vi "lab1.vi"() -> ()   [LabVIEW 2025]
panel:
  out "Decoder":bool[][](array[boolean])
  in  "CRC":bool[](array[boolean])
  out "Encoder":bool[][](array[boolean])
  in  "In":bool[](array[boolean])
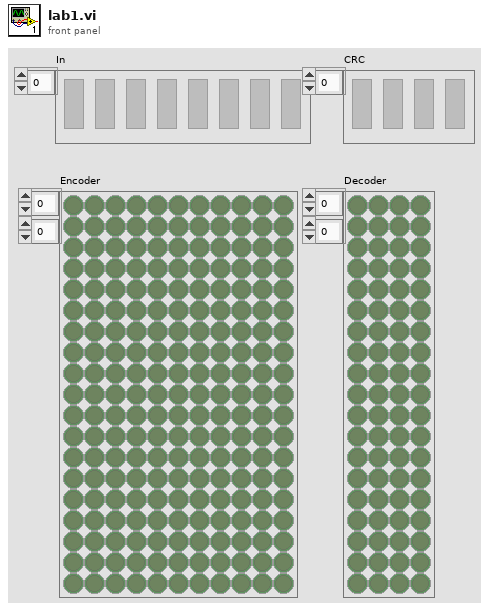
[diagram p1: front panel]
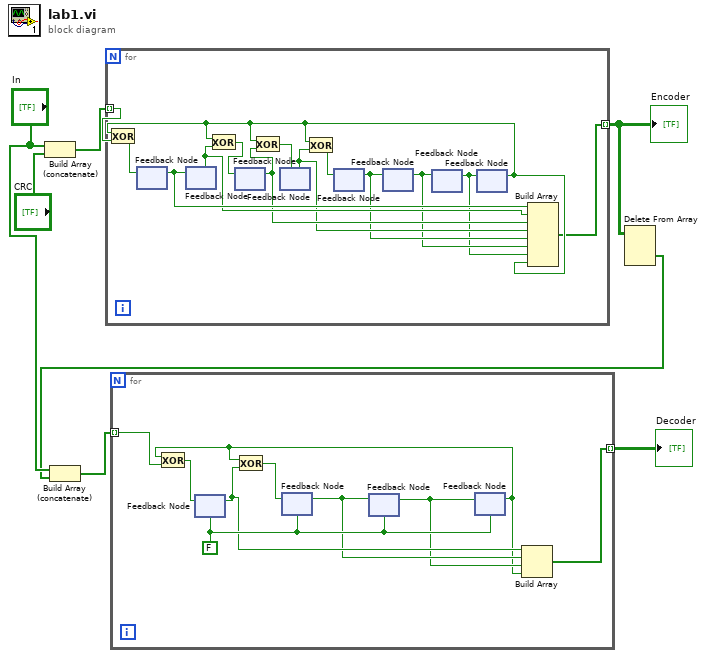
[diagram p0: block diagram]
diagram:
  n1 = Build Array (concatenate)("In", "CRC") -> (w6:bool[])
  n2 = for {
    tunnel: w6 -> [w17] mode=indexing
    tunnel: [w8] -> w2 mode=indexing
    n3 = feedback #1() -> (w16:bool)  [unwired: 1 in]
    n4 = feedback #2() -> (w15:bool)  [unwired: 1 in]
    n5 = feedback-in #2(w16) -> ()
    n6 = feedback #3() -> (w14:bool)  [unwired: 1 in]
    n7 = feedback #4() -> (w13:bool)  [unwired: 1 in]
    n8 = feedback #5() -> (w12:bool)  [unwired: 1 in]
    n9 = feedback #6() -> (w11:bool)  [unwired: 1 in]
    n10 = feedback-in #6(w12) -> ()
    n11 = feedback #7() -> (w10:bool)  [unwired: 1 in]
    n12 = feedback-in #7(w11) -> ()
    n13 = feedback #8() -> (w9:bool)  [unwired: 1 in]
    n14 = Exclusive Or(1:w17, 2:w9) -> (0:w21:bool)
    n15 = feedback-in #1(w21) -> ()
    n16 = Exclusive Or(1:w15, 2:w9) -> (0:w20:bool)
    n17 = feedback-in #3(w20) -> ()
    n18 = Exclusive Or(1:w14, 2:w9) -> (0:w19:bool)
    n19 = feedback-in #4(w19) -> ()
    n20 = Exclusive Or(1:w13, 2:w9) -> (0:w18:bool)
    n21 = feedback-in #5(w18) -> ()
    n22 = feedback-in #8(w10) -> ()
    n23 = Build Array(w16, w15, w14, w13, w12, w11, w10, w9) -> (w8:bool[])
  }
  "Encoder" <- w2
  n24 = Delete From Array(array=w2) -> (deleted portion=w1:bool[])  [unwired: 3 in, 1 out]
  n25 = Build Array (concatenate)("In", w1) -> (w4:bool[])
  n26 = for {
    tunnel: w4 -> [w27] mode=indexing
    tunnel: [w22] -> w5 mode=indexing
    w28 = FALSE
    n27 = feedback #9(w28) -> (w26:bool)
    n28 = feedback #10(w28) -> (w25:bool)
    n29 = feedback #11(w28) -> (w24:bool)
    n30 = feedback-in #11(w25) -> ()
    n31 = feedback #12(w28) -> (w23:bool)
    n32 = Exclusive Or(1:w27, 2:w23) -> (0:w30:bool)
    n33 = feedback-in #9(w30) -> ()
    n34 = Exclusive Or(1:w26, 2:w23) -> (0:w29:bool)
    n35 = feedback-in #10(w29) -> ()
    n36 = feedback-in #12(w24) -> ()
    n37 = Build Array(w26, w25, w24, w23) -> (w22:bool[])
  }
  "Decoder" <- w5
